vi "Pulse train.vi"(6 "Reverse?":bool, 8 "Total length":i32, 9 "Cycles":i32, 10 "Cycle length":i32, 11 "Pulse length":i32) -> (2 "output array":u8[](array[numeric]))   [LabVIEW 2020, in "Scan Generators.lvlib"]
uses:
  Scan Generators.lvlib
panel:
  out "Waveform Graph":u8[](graph)
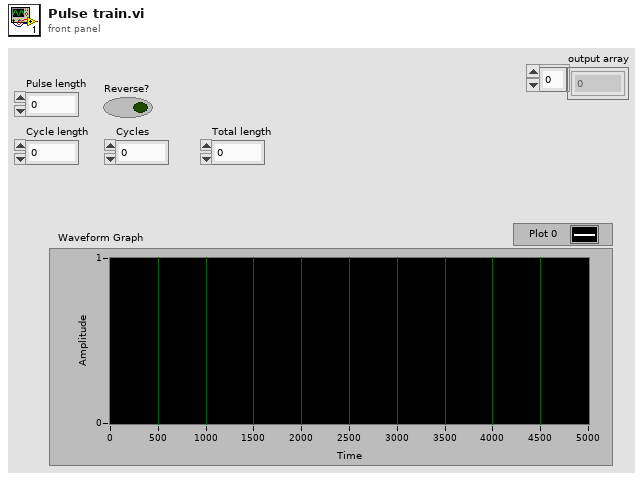
[diagram p1: front panel]
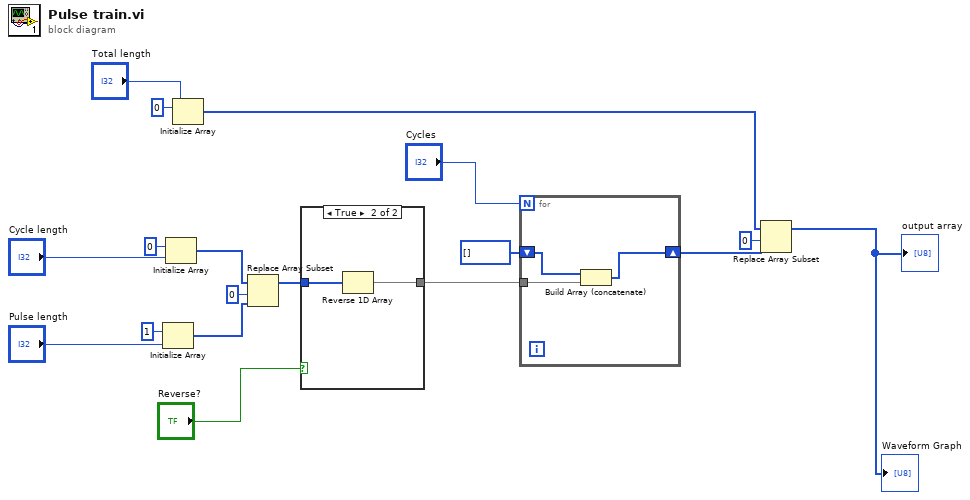
[diagram p0: block diagram]
diagram:
  n1 = Initialize Array(u8 1 ("element"), "Pulse length") -> (w13:u8[])
  n2 = Initialize Array(u8 0 ("element"), "Cycle length") -> (w12:u8[])
  n3 = Initialize Array(u8 0 ("element"), "Total length") -> (w2:u8[])
  n4 = Replace Array Subset(array=w12, new element=w13, index=0) -> (w10:u8[])
  n5 = case shown="True" "Reverse?" {
    tunnel: w10 -> [w19 w21]
    tunnel: [w19 w20] -> w8
    frame False {
    }
    frame True {
      n6 = Reverse 1D Array(array=w21) -> (reversed array=w20:u8[])
    }
  }
  n7 = for {
    N: "Cycles" -> [_]
    tunnel: w8 -> [w24]
    shift-right: [w23] -> w3
    shift-left: u8[] [] -> [w22]
    n8 = Build Array (concatenate)(w22, w24) -> (w23:u8[])
  }
  n9 = Replace Array Subset(array=w2, new element=w3, index=0) -> (→"Waveform Graph" →"output array":u8[])
